vi "ASD HIS BIN.vi"(8 "bin length":dbl=0.05 format="%#_13g", 10 "min":dbl=-0.175 format="%#_13g", 11 "MAX":dbl) -> (0 "New bin":dbl, 2 "New MIN":dbl, 3 "New MAX":dbl)   [LabVIEW 2018]
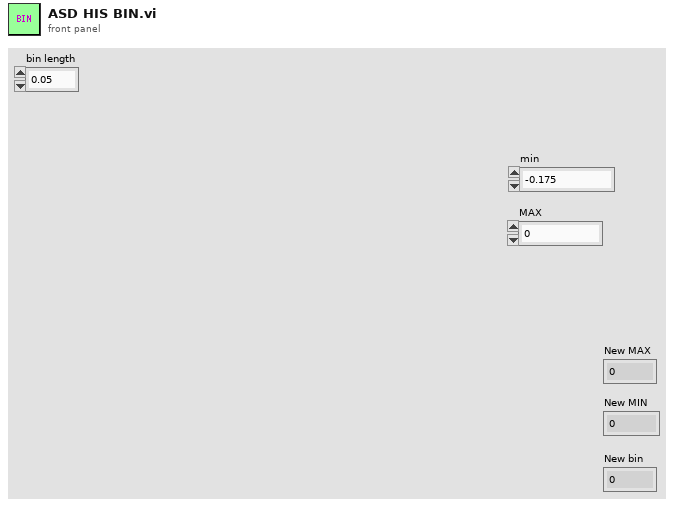
[diagram p1: front panel]
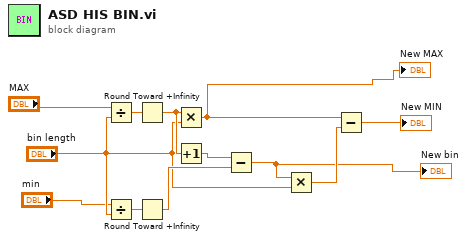
[diagram p0: block diagram]
diagram:
  n1 = Divide(x="MAX", y="bin length") -> (x/y=w12:dbl)
  n2 = Divide(x="min", y="bin length") -> (x/y=w10:dbl)
  n3 = Round Toward +Infinity(x=w12) -> (ceil(x): smallest int >= x=w11:dbl)
  n4 = Round Toward +Infinity(x=w10) -> (ceil(x): smallest int >= x=w8:dbl)
  n5 = Multiply(x=w11, y="bin length") -> (x*y=w3:dbl)
  "New MAX" <- w3
  n6 = Increment(x=w11) -> (x+1=w9:dbl)
  n7 = Subtract(x=w9, y=w8) -> (x-y=w1:dbl)
  "New bin" <- w1
  n8 = Multiply(x=w1, y="bin length") -> (x*y=w7:dbl)
  n9 = Subtract(x=w3, y=w7) -> (x-y=→"New MIN":dbl)
